vi "Build_Asylum_GetGroupLabels.vi"(8 "error in (no error)":errorcluster, 10 "textWave":string, 11 "groupName":string) -> (0 "error out":errorcluster, 3 "Command":string)   [LabVIEW 2019]
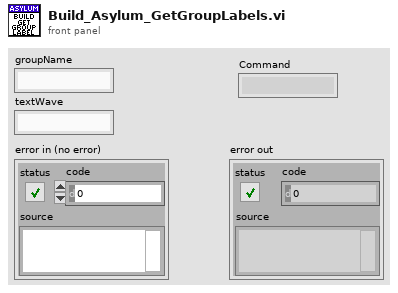
[diagram p1: front panel]
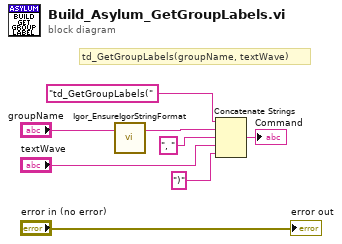
[diagram p0: block diagram]
diagram:
  # "td_GetGroupLabels(groupName, textWave)"
  n1 = call <userlib>:"Igor_EnsureIgorStringFormat.vi"("Value"="groupName") -> ("Value"=w3:string)  [unwired: 2 in]
  n2 = Concatenate Strings("td_GetGroupLabels(", w3, ", " ("string"), "textWave", ")" ("string")) -> (→"Command":string)
  "error out" <- "error in (no error)"
